vi "GetCacheFile.vi"(8 "error in (no error)":errorcluster, 10 "feed GUID":string) -> (0 "error out":errorcluster, 3 "cache file":path)   [LabVIEW 2023, in "GettingStartedWindow.lvlib" / "Feed_link.lvclass"]
uses:
  <resource>/modes/FRC/GSW/Classes/Feed_link/Feed_link.lvclass
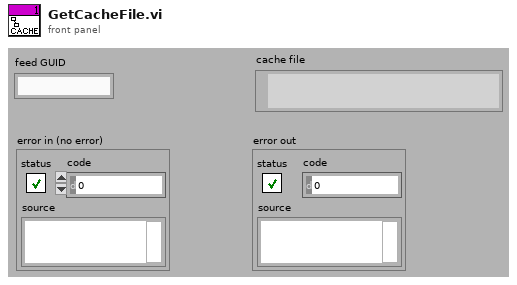
[diagram p1: front panel]
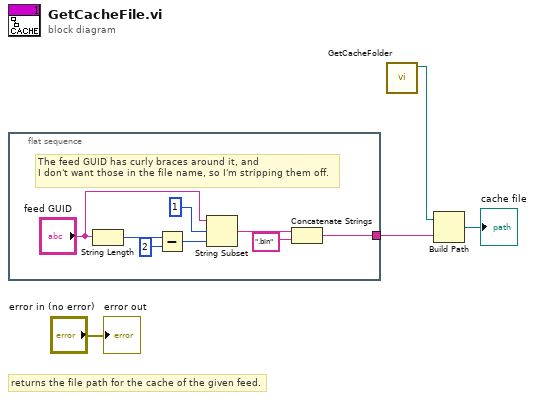
[diagram p0: block diagram]
diagram:
  # "returns the file path for the cache of the given feed."
  n1 = flat-sequence {
    tunnel: [w11] -> w3
    frame #0 {
      # "The feed GUID has curly braces around it, and \nI don't want those in the file name, so I'm stripping them off."
      n2 = String Length(string="feed GUID") -> (length=w9:i32)
      n3 = Subtract(x=w9, y=2) -> (x-y=w7:i32)
      n4 = String Subset(string="feed GUID", offset (0)=1, length (rest)=w7) -> (substring=w5:string)
      n5 = Concatenate Strings(w5, ".bin" ("string")) -> (w11:string)
    }
  }
  n6 = call <resource>:"GetCacheFolder.vi"() -> ("cache folder"=w4:path)  [unwired: 1 in, 10 out]
  n7 = Build Path(base path=w4, name or relative path=w3) -> (appended path=→"cache file":path)
  "error out" <- "error in (no error)"
